vi "niGPS Streaming File (5671).vi"(9 "GPS Binary File Path":path=path "C:/Program Files/National Instruments/GPS/Mt Everest.bin") -> ()   [LabVIEW 2025]
doc: "This example shows how to generate a GPS signal by streaming from a GPS binary file. This example uses two separate instrument handles: the Upconverter Resource Name and the Arbitrary Waveform Generator (AWG) Resource Name."
uses:
  <vilib>/RF Toolkits/GPS/Controls/gps version control.ctl
panel:
  out "Generating":bool
  in  "Stop":bool
  out "Space Available in Streaming Waveform (S)":i32(slide) scale=-1.0..20971520.0
  out "number of elements read":u32
  out "Total Number of Samples":u32
  in  "AWG Resource Name":refnum<k15>="Dev1"
  in  "Upconverter \nResource Name":refnum<k15>="Dev2" caption="resource name"
  out "Error Out":errorcluster
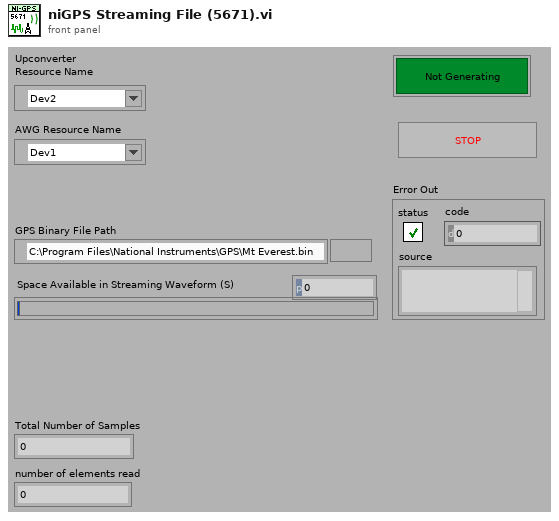
[diagram p1: front panel]
types:
  T1 = typedef "gps version control.ctl" = i32
  T2 = enum16{"open", "replace", "create", "open or create", "replace or create", "replace or create with confirmation"}
  T3 = typedef "gpsv1_refnum.ctl" = refnum<k20>
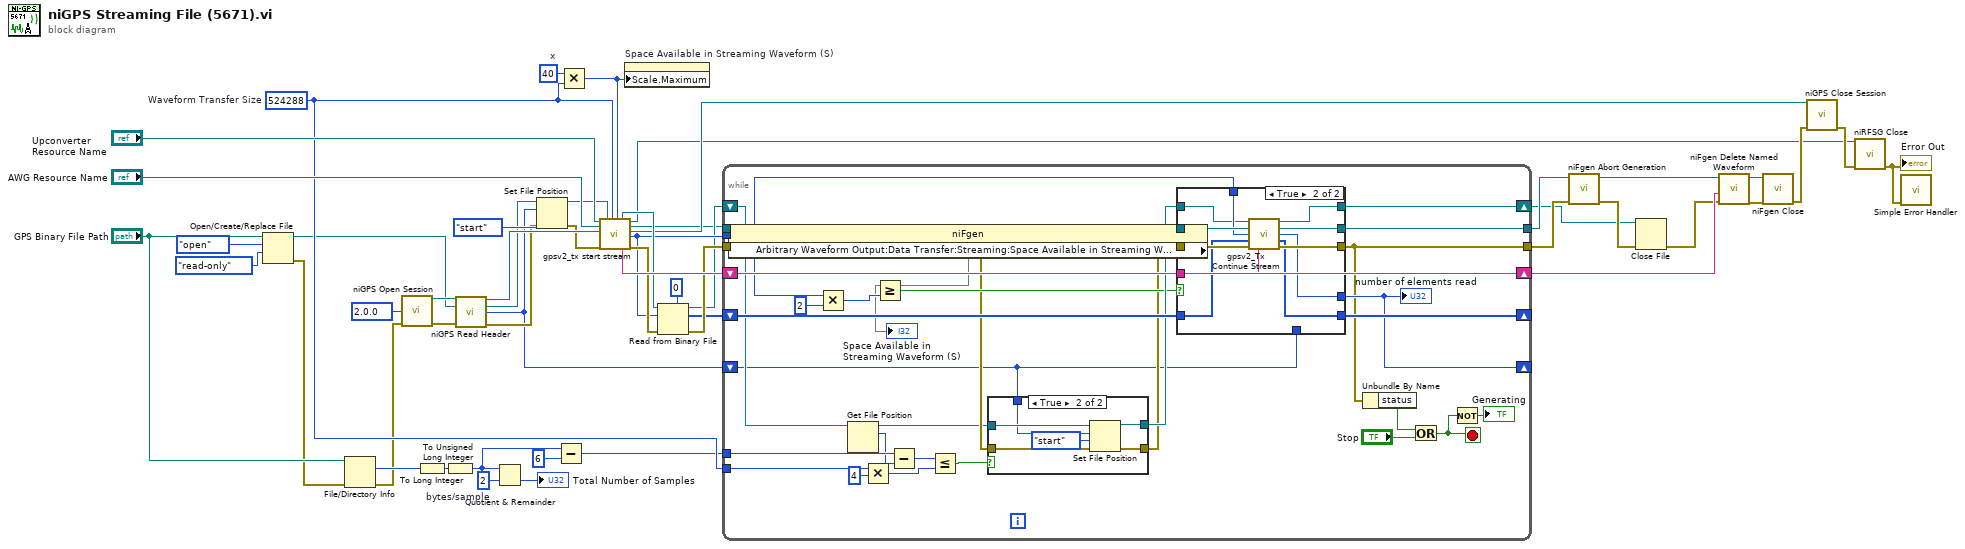
[diagram p0: block diagram]
diagram:
  w1 = T1 20000 items=["2.0.0"=20000] ("toolkit compatibility version")
  w25 = u32 524288  # Waveform Transfer Size
  w41 = u32 2  # bytes/sample
  w43 = u32 40  # x
  n1 = Open/Create/Replace File(file path (use dialog)="GPS Binary File Path", operation (0:open)=T2."open", access (0:read/write)=enum16{"read/write", "read-only", "write-only"}."read-only") -> (refnum out=w2:refnum<file>, error out=w7:errorcluster)  [unwired: 1 in, 3 out]
  n2 = File/Directory Info(path="GPS Binary File Path", error in=w7) -> (size=w38:i64, error out=w6:errorcluster)  [unwired: 5 out]
  n3 = call <vilib>:"niGPS Open Session.vi"("toolkit compatibility version"=w1, "error in"=w6) -> ("nigps session out"=w3:T3, "error out"=w4:errorcluster)  [unwired: 1 in, 11 out]
  n4 = To Long Integer(number=w38) -> (32bit integer=w42:i32)
  n5 = To Unsigned Long Integer(number=w42) -> (unsigned 32bit integer=w39:u32)
  n6 = call <vilib>:"niGPS Read Header.vi"("nigps session"=w3, "file refnum"=w2, "error in"=w4) -> ("nigps session out"=w24:T3, "file refnum out"=w14:refnum<file>, "data offset (bytes)"=w5:i64, "error out"=w13:errorcluster)  [unwired: 9 out]
  n7 = Quotient & Remainder(x=w39, y=w41) -> (floor(x/y)=→"Total Number of Samples":u32)  [unwired: 1 out]
  n8 = Set File Position(offset (in bytes) (0)=w5, refnum=w14, from (0:start)=enum16{"start", "end", "current"}."start", error in=w13) -> (refnum out=w16:refnum<file>, error out=w12:errorcluster)
  n9 = Subtract(x=w39, y=u32 6) -> (x-y=w20:u32)
  n10 = Multiply(x=w43, y=w25) -> (x*y=w11:u32)
  n11 = call "gpsv2_tx start stream.vi"("UPC Resource Name"="Upconverter \nResource Name", "AWG Resource Name"="AWG Resource Name", "nigps session"=w24, "error in"=w12, "refnum in"=w16, "Waveform Transfer Size"=w25, "onboard StreamingWaveform Size"=w11) -> ("refnum out"=w34:refnum<file>, "Waveform Name Out"=w48:string, "UPC handle"=w18:refnum<k15>, "AWG Handle"=w17:refnum<k15>, "nigps session out"=w23:T3, "Waveform Transfer Size (samples)"=w33:u32, "error out"=w37:errorcluster)  [unwired: 6 out]
  n12 = property on="Space Available in Streaming Waveform (S)" class="Slide (strict)"("Scale.Maximum"=w11) -> ()  [unwired: 2 in, 2 out]
  n13 = Read from Binary File(5:i16 0 ("element"), 8:w37, 10:w33, 11:w34) -> (0:w36:errorcluster, 2:w31:i16[], 3:w32:refnum<file>)  [unwired: 3 out]
  n14 = while {
    tunnel: w33 -> [w65]
    tunnel: [w72] -> w46
    tunnel: [w82] -> w45
    tunnel: w17 -> [w81]
    tunnel: w36 -> [w78]
    shift-right: [w79] -> w44
    shift-left: w48 -> [w79]
    shift-right: [w76] -> _
    shift-left: w31 -> [w77]
    shift-right: [w83] -> w28
    shift-left: w32 -> [w61]
    shift-right: [w75] -> _
    shift-left: w5 -> [w56]
    tunnel: w20 -> [w67]
    tunnel: w25 -> [w57]
    stop <- w53 stop-if-true
    n15 = property class="niFgen"(reference=w81, error in=w78) -> (reference out=w80:refnum<k15>, error out=w69:errorcluster, "Arbitrary Waveform Output:Data Transfer:Streaming:Space Available in Streaming Waveform"=w55)
    "Space Available in Streaming Waveform (S)" <- w55
    n16 = Multiply(x=w65, y=u32 2) -> (x*y=w64:u32)
    n17 = Get File Position(7:w61) -> (2:w63:i64, 3:w62:refnum<file>)  [unwired: 1 in, 1 out]
    n18 = Multiply(x=w57, y=u32 4) -> (x*y=w58:u32)
    n19 = Greater Or Equal?(x=w55, y=w64) -> (x >= y?=w73:bool)
    n20 = Subtract(x=w67, y=w63) -> (x-y=w70:i64)
    n21 = Less Or Equal?(x=w70, y=w58) -> (x <= y?=w60:bool)
    n22 = case shown="True" w60 {
      tunnel: w62 -> [w85 w90]
      tunnel: [w85 w91] -> w74
      tunnel: w69 -> [w84 w89]
      tunnel: [w84 w88] -> w68
      tunnel: w56 -> [_ w87]
      frame False {
      }
      frame True {
        n23 = Set File Position(offset (in bytes) (0)=w87, refnum=w90, from (0:start)=enum16{"start", "end", "current"}."start", error in=w89) -> (refnum out=w91:refnum<file>, error out=w88:errorcluster)
      }
    }
    n24 = case shown="True" w73 {
      tunnel: w74 -> [w96 w99]
      tunnel: [w96 w98] -> w83
      tunnel: [w94 w107] -> w72
      tunnel: [w95 w106] -> w82
      tunnel: w80 -> [w95 w105]
      tunnel: w79 -> [_ w104]
      tunnel: w65 -> [_ w103]
      tunnel: w68 -> [w94 w102]
      tunnel: w77 -> [w93 w100]
      tunnel: [w93 w101] -> w76
      tunnel: [w92 w97] -> w75
      tunnel: w56 -> [w92 _]
      frame False {
      }
      frame True {
        n25 = call "gpsv2_Tx Continue Stream.vi"("refnum in"=w99, "AWG Handle in"=w105, "Transfer size (samples)"=w103, "data in"=w100, "error in"=w102, "Waveform Name"=w104) -> ("refnum out"=w98:refnum<file>, "AWG handle out"=w106:refnum<k15>, "no. of elements read"=w97:i64, "data out"=w101:i16[], "error out"=w107:errorcluster)  [unwired: 5 out]
      }
    }
    "number of elements read" <- w75
    n26 = Unbundle By Name(w72) -> ("status"=w71:bool)
    n27 = Or(x=w71, y="Stop") -> (x .or. y?=w53:bool)
    n28 = Not(x=w53) -> (.not. x?=→"Generating":bool)
  }
  n29 = call <instrlib>:"niFgen Abort Generation.vi"("error in (no error)"=w46, "Instrument Handle"=w45) -> ("error out"=w30:errorcluster, "Instrument Handle Out"=w47:refnum<k15>)  [unwired: 8 out]
  n30 = Close File(refnum=w28, error in=w30) -> (error out=w29:errorcluster)  [unwired: 1 out]
  n31 = call <instrlib>:"niFgen Delete Named Waveform.vi"("error in (no error)"=w29, "Waveform Name"=w44, "Instrument Handle"=w47) -> ("error out"=w51:errorcluster, "Instrument Handle Out"=w50:refnum<k15>)  [unwired: 1 in, 6 out]
  n32 = call <instrlib>:"niFgen Close.vi"("error in (no error)"=w51, "Instrument Handle"=w50) -> ("error out"=w22:errorcluster)  [unwired: 9 out]
  n33 = call <vilib>:"niGPS Close Session.vi"("nigps session"=w23, "error in"=w22) -> ("error out"=w21:errorcluster)  [unwired: 13 out]
  n34 = call <instrlib>:"niRFSG Close.vi"("instrument handle"=w18, "error in"=w21) -> ("error out"=w49:errorcluster)  [unwired: 13 out]
  "Error Out" <- w49
  n35 = call <vilib>:"Simple Error Handler.vi"("error in (no error)"=w49) -> ()  [unwired: 1 in, 8 out]
